vi "Add Case Structure Frame (by Name).vi"(8 "error in (no error)":errorcluster, 10 "Frame name":string, 11 "CaseStructure in":refnum<vi>) -> (0 "error out":errorcluster, 2 "Case Frame":refnum<vi>, 3 "CaseStructure out":refnum<vi>)   [LabVIEW 2019, in "gRPC Template Creation Utility.lvlib"]
uses:
  gRPC Template Creation Utility.lvlib
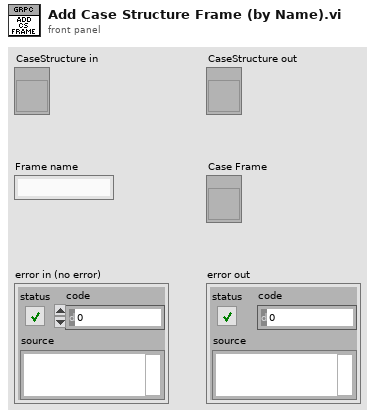
[diagram p1: front panel]
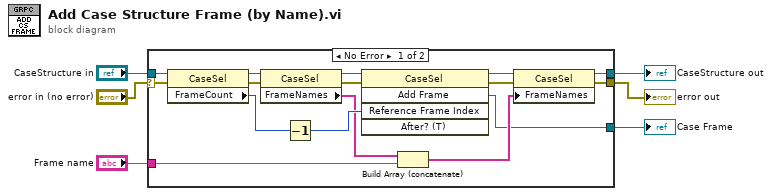
[diagram p0: block diagram]
diagram:
  n1 = case shown="No Error" "error in (no error)" {
    selector: "error in (no error)" -> [w15 w24]
    tunnel: [w16 w23] -> w6
    tunnel: [w13 w24] -> w5
    tunnel: "CaseStructure in" -> [w18 w23]
    tunnel: "Frame name" -> [w19 _]
    tunnel: [w7 _] -> w1
    frame No Error {
      n2 = property class="CaseSel"(reference=w18, error in=w15) -> (reference out=w12:refnum<vi>, error out=w11:errorcluster, "FrameCount"=w22:i32)
      n3 = property class="CaseSel"(reference=w12, error in=w11) -> (reference out=w9:refnum<vi>, error out=w10:errorcluster, "FrameNames"=w8:string[])
      n4 = Decrement(x=w22) -> (x-1=w21:i32)
      n5 = invoke class="CaseSel" method="Add Frame"(reference=w9, error in=w10, "Reference Frame Index"=w21) -> (reference out=w17:refnum<vi>, error out=w14:errorcluster, "Add Frame"=w7:refnum<vi>)  [unwired: 2 in, 2 out]
      n6 = Build Array (concatenate)(w8, w19) -> (w20:string[])
      n7 = property class="CaseSel"(reference=w17, error in=w14, "FrameNames"=w20) -> (reference out=w16:refnum<vi>, error out=w13:errorcluster)
    }
    frame Error {
    }
  }
  "error out" <- w5
  "CaseStructure out" <- w6
  "Case Frame" <- w1
